vi "Acquire Data.vi"(7 "user event":T2, 8 "error in (no error)":errorcluster, 9 "UI Refs":T1, 10 "Waveforms":waveform(dbl)[](array[waveform]), 11 "H1 Frequency Response":refnum<class "H1 Frequency Response.lvclass">) -> (0 "error out":errorcluster, 3 "H1 Frequency Response out":refnum<class "H1 Frequency Response.lvclass">)   [LabVIEW 2025, in "H1 Plotter.lvlib" / "H1 Frequency Response.lvclass"]
uses:
  H1 Frequency Response.lvclass
  Users/Public/Documents/Sandia National Labs/TSS Plugin/CEF.lvlibp/Node/UserEventRef.ctl
  Users/Public/Documents/Sandia National Labs/TSS Plugin/Tests/XY Plotter.lvlibp/XY Plotter configuration/Read XY Plotter.vi
  Users/Public/Documents/Sandia National Labs/TSS Plugin/CEF.lvlibp/serializable configuration/CEF_serializable configuration.lvclass
  H1 Frequency Response.lvclass/H1 Frequency Response.ctl
  Users/Public/Documents/Sandia National Labs/TSS Plugin/Tests/XY Plotter.lvlibp/XY  Plotter/Timing FGV.vi
  Users/Public/Documents/Sandia National Labs/TSS Plugin/Tests/XY Plotter.lvlibp/XY  Plotter/XY Plotter.lvclass
  Users/Public/Documents/Sandia National Labs/TSS Plugin/CEF.lvlibp/Node/CEF_Node.lvclass
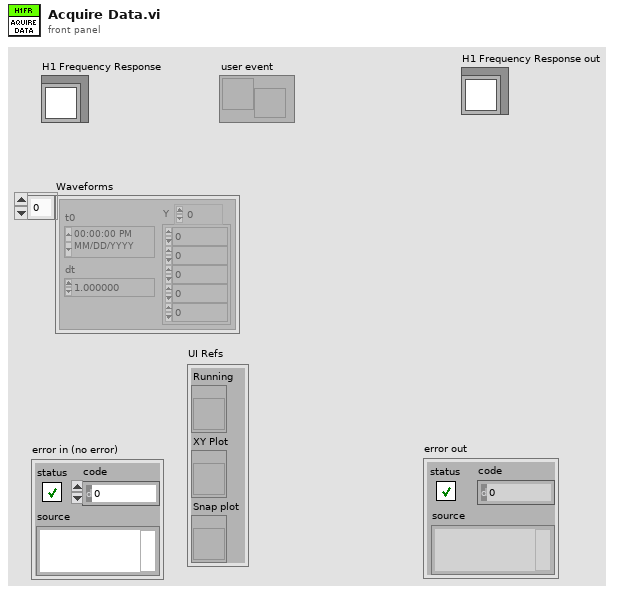
[diagram p1: front panel]
types:
  T1 = cluster{"Running":refnum<vi>, "XY Plot":refnum<vi>, "Snap plot":refnum<vi>}
  T2 = typedef "CEF.lvlibp/CEF_Node.lvclass/UserEventRef.ctl" = refnum<user-event>
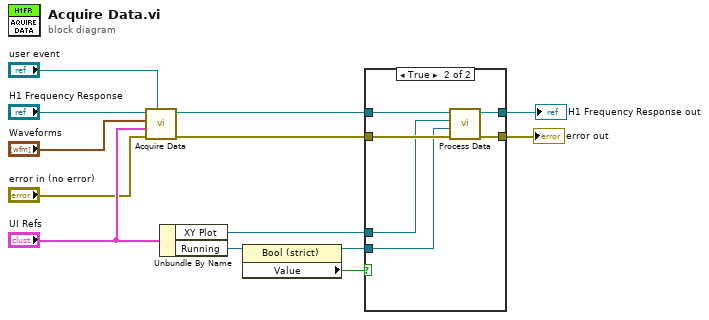
[diagram p0: block diagram]
diagram:
  n1 = call-parent "Acquire Data.vi"("user event"="user event", "error in (no error)"="error in (no error)", "UI Refs"="UI Refs", "Waveforms"="Waveforms", "XY Plotter"="H1 Frequency Response") -> ("error out"=w1:errorcluster, "XY Plotter out"=w6:refnum<class "H1 Frequency Response.lvclass">)  [unwired: 5 in]
  n2 = Unbundle By Name("UI Refs") -> ("XY Plot"=w8:refnum<vi>, "Running"=w9:refnum<vi>)
  n3 = property class="Bool (strict)"(reference=w9) -> (reference out=w12:refnum<vi>, "Value"=w13:bool)  [unwired: 1 in, 1 out]
  n4 = case shown="True" w13 {
    tunnel: [w15 w21] -> w11
    tunnel: w12 -> [_ w16]
    tunnel: w6 -> [w15 w20]
    tunnel: [w14 w19] -> w10
    tunnel: w8 -> [_ w17]
    tunnel: w1 -> [w14 w18]
    frame False {
    }
    frame True {
      n5 = call "Process Data.vi"("error in (no error)"=w18, "Running"=w16, "XY Plot"=w17, "H1FR"=w20) -> ("error out"=w19:errorcluster, "H1FR out"=w21:refnum<class "H1 Frequency Response.lvclass">)  [unwired: 6 in]
    }
  }
  "error out" <- w10
  "H1 Frequency Response out" <- w11
